vi "FuncVI_Sub - vhShow - Launcher.vi"(7 "VC Handle":T1=-1, 8 "error in":errorcluster, 9 "left-top corner":cluster{"x":i16, "y":i16}={"x"=-1, "y"=-1}, 10 "win name":string, 11 "var name":string) -> (0 "error out":errorcluster)   [LabVIEW 2021]
doc: "::: CalcExpress Toolkit :::\nCopyright (c) 2000-2026 Konstantin Shifershteyn. All rights reserved."
uses:
  cetypes.llb/VarMan Variable Context Handle.ctl
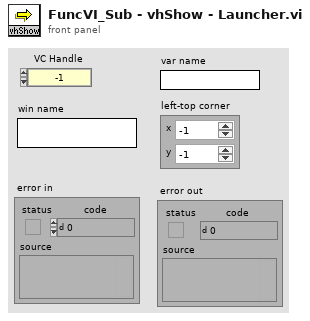
[diagram p1: front panel]
types:
  T1 = typedef "VarMan Variable Context Handle.ctl" = i32
  T2 = enum32{"Invalid", "Standard", "Closed", "Hidden", "Minimized", "Maximized"}
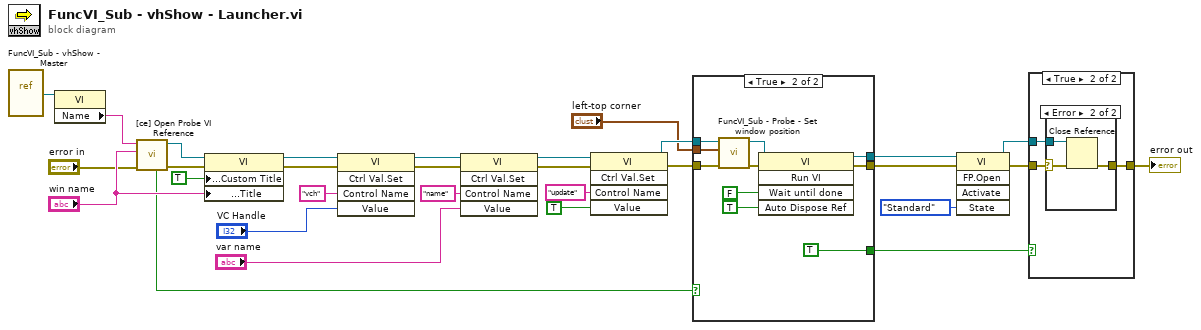
[diagram p0: block diagram]
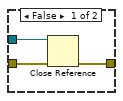
[diagram p2: hidden frame]
diagram:
  n1 = vi-ref "FuncVI_Sub - vhShow - Master.vi"() -> (w6:refnum<vi>)
  n2 = property class="VI"(reference=w6) -> ("Name"=w5:string)  [unwired: 1 in, 2 out]
  n3 = call "[ce] Open Probe VI Reference.vi"("error in"="error in", "VI instance name"="win name", "master VI name"=w5) -> ("error out"=w15:errorcluster, "vi refnum"=w14:refnum<vi>, "new window?"=w12:bool)  [unwired: 6 in]
  n4 = property class="VI"(reference=w14, error in=w15, "Front Panel Window:Custom Title"=TRUE ("Front Panel.CustomTitle"), "Front Panel Window:Title"="win name") -> (reference out=w17:refnum<vi>, error out=w16:errorcluster)
  n5 = invoke class="VI" method="Ctrl Val.Set"(reference=w17, error in=w16, "Control Name"="vch", "Value"="VC Handle") -> (reference out=w19:refnum<vi>, error out=w18:errorcluster)  [unwired: 1 in, 3 out]
  n6 = invoke class="VI" method="Ctrl Val.Set"(reference=w19, error in=w18, "Control Name"="name", "Value"="var name") -> (reference out=w25:refnum<vi>, error out=w24:errorcluster)  [unwired: 1 in, 3 out]
  n7 = invoke class="VI" method="Ctrl Val.Set"(reference=w25, error in=w24, "Control Name"="update", "Value"=TRUE) -> (reference out=w23:refnum<vi>, error out=w22:errorcluster)  [unwired: 1 in, 3 out]
  n8 = case shown="True" w12 {
    tunnel: [w32 w40] -> w29
    tunnel: [w31 w41] -> w28
    tunnel: w23 -> [w32 w36]
    tunnel: w22 -> [w31 w39]
    tunnel: [_ TRUE] -> w2
    tunnel: "left-top corner" -> [_ w33]
    frame False {
    }
    frame True {
      n9 = call "FuncVI_Sub - Probe - Set window position.vi"("error in"=w39, "left-top corner"=w33, "VI RefNum"=w36) -> ("error out"=w38:errorcluster, "dup VI Refnum"=w37:refnum<vi>)  [unwired: 7 in]
      n10 = invoke class="VI" method="Run VI"(reference=w37, error in=w38, "Wait until done"=FALSE, "Auto Dispose Ref"=TRUE ("Auto Dispose Reference")) -> (reference out=w40:refnum<vi>, error out=w41:errorcluster)  [unwired: 1 in, 3 out]
    }
  }
  n11 = invoke class="VI" method="FP.Open"(reference=w29, error in=w28, "State"=T2."Standard") -> (reference out=w30:refnum<vi>, error out=w4:errorcluster)  [unwired: 2 in, 3 out]
  n12 = case shown="True" w2 {
    tunnel: w30 -> [w44 w48]
    tunnel: w4 -> [w45 w47]
    tunnel: [w43 w46] -> w3
    frame False {
      n13 = Close Reference(reference=w44, error in (no error)=w45) -> (error out=w43:errorcluster)
    }
    frame True {
      n14 = case shown="Error" w47 {
        selector: w47 -> [w49 w51]
        tunnel: w48 -> [_ w52]
        tunnel: [w49 w50] -> w46
        frame No Error {
        }
        frame Error {
          n15 = Close Reference(reference=w52, error in (no error)=w51) -> (error out=w50:errorcluster)
        }
      }
    }
  }
  "error out" <- w3
